vi "[ce] Get LV Memory Use.vi"() -> (2 "MemStats":T1, 3 "Total KB Allocated":u64)   [LabVIEW 2021]
doc: "::: CalcExpress Toolkit :::\nCopyright (c) 2000-2026 Konstantin Shifershteyn. All rights reserved."
uses:
  cersrc/celveng32.dll
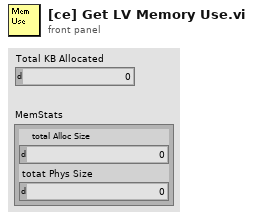
[diagram p1: front panel]
types:
  T1 = cluster{"total Alloc Size":u64, "totat Phys Size":u64}
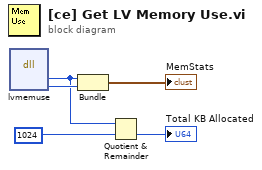
[diagram p0: block diagram]
diagram:
  n1 = dll-call lib="C:/LV Projects/CalcExpress 40 LV2021/vi.lib/addons/CalcExpress/cersrc/celveng*.dll" fn="lvmemuse"() -> ("totAllocSize"=w3:u64, "totPhysSize"=w5:u64)  [unwired: 6 in, 2 out]
  n2 = Bundle("totAllocSize"=w3, "totPhysSize"=w5) -> (→"MemStats":cluster{"totAllocSize":u64, "totPhysSize":u64})  [unwired: 1 in]
  n3 = Quotient & Remainder(x=w3, y=u64 1024) -> (floor(x/y)=→"Total KB Allocated":u64)  [unwired: 1 out]
